vi "random.vi"(8 "error in (no error)":errorcluster, 9 "min":i32, 10 "max":i32) -> (0 "error out":errorcluster, 2 "random":i32)   [LabVIEW 2018, in "ThirdPartyYoutubeClass.lvclass"]
uses:
  ThirdPartyYoutubeClass.lvclass
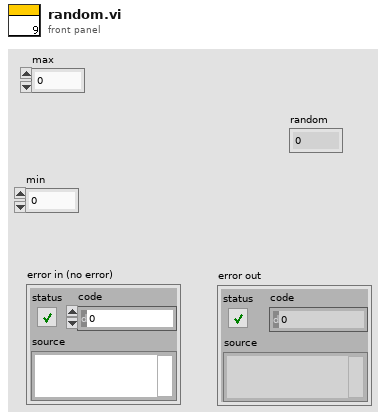
[diagram p1: front panel]
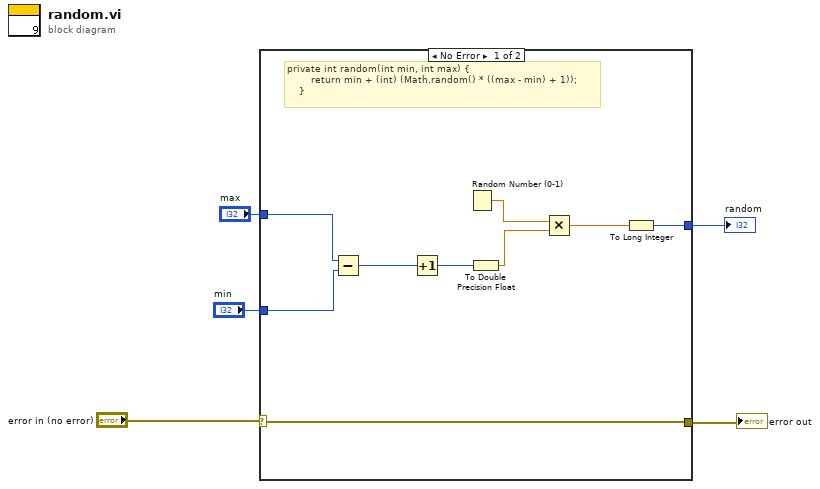
[diagram p0: block diagram]
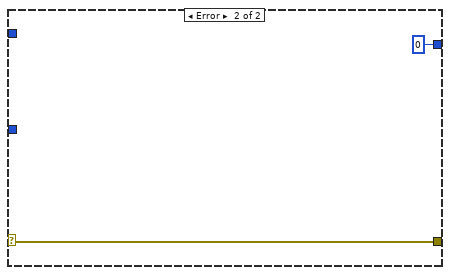
[diagram p2: hidden frame]
diagram:
  n1 = case shown="No Error" "error in (no error)" {
    selector: "error in (no error)" -> [w6 w16]
    tunnel: "max" -> [w14 _]
    tunnel: "min" -> [w13 _]
    tunnel: [w7 0] -> w3
    tunnel: [w6 w16] -> w1
    frame No Error {
      # "private int random(int min, int max) {\n        return min + (int) (Math.random() * ((max - min) + 1));\n    }"
      n2 = Subtract(x=w14, y=w13) -> (x-y=w12:i32)
      n3 = Increment(x=w12) -> (x+1=w10:i32)
      n4 = Random Number (0-1)() -> (number: 0 to 1=w11:dbl)
      n5 = To Double Precision Float(number=w10) -> (double precision float=w9:dbl)
      n6 = Multiply(x=w11, y=w9) -> (x*y=w8:dbl)
      n7 = To Long Integer(number=w8) -> (32bit integer=w7:i32)
    }
    frame Error {
    }
  }
  "random" <- w3
  "error out" <- w1
